vi "展开空白块.vi"(1 "索引":i32, 2 "地图":i16[][](array[numeric])) -> (0 "输出地图":i16[][](array[numeric]))   [LabVIEW 2017]
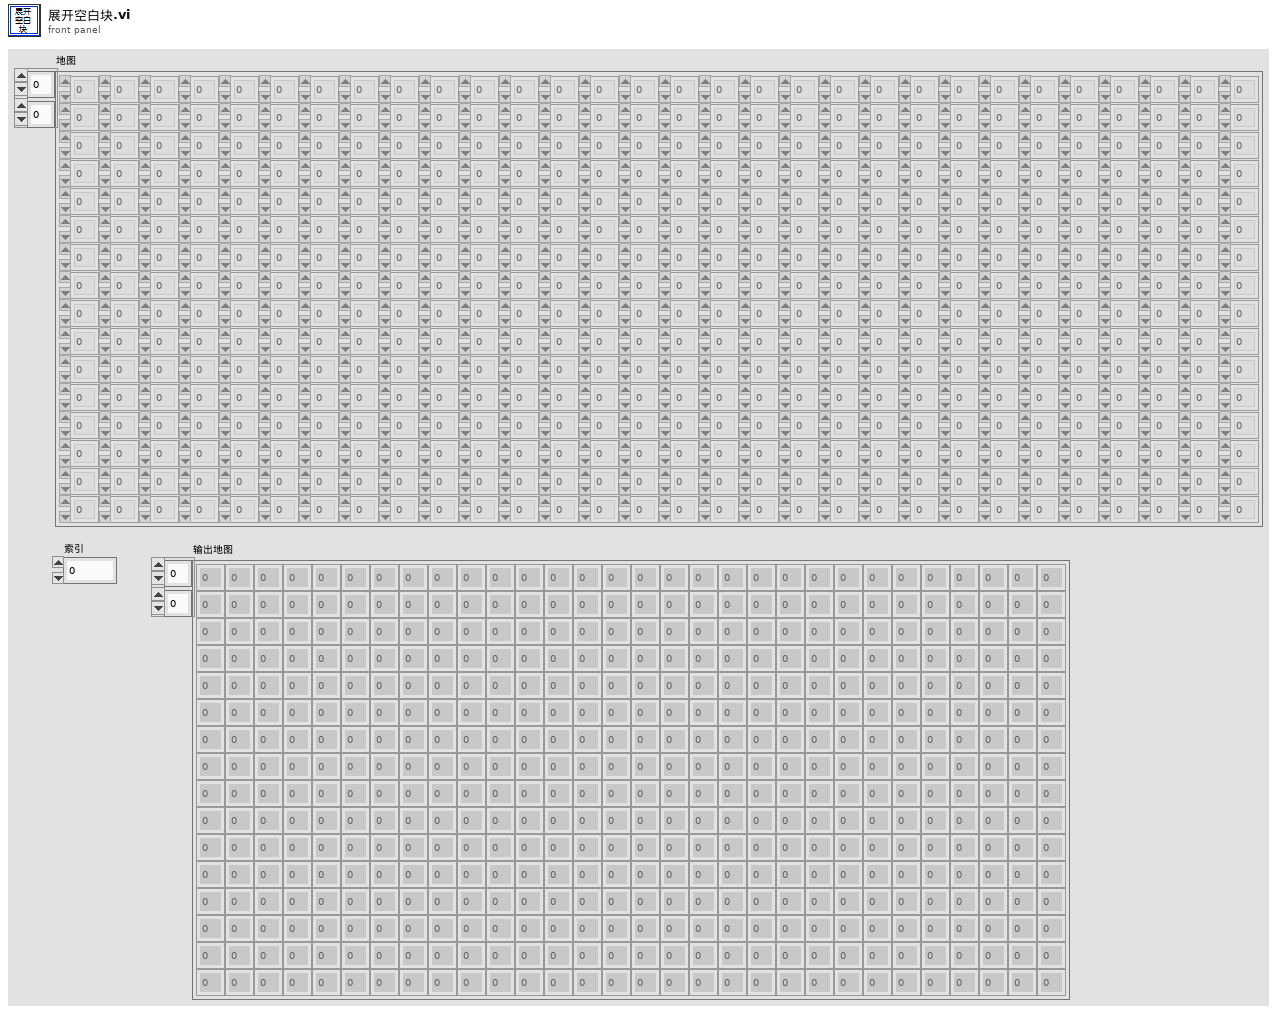
[diagram p1: front panel]
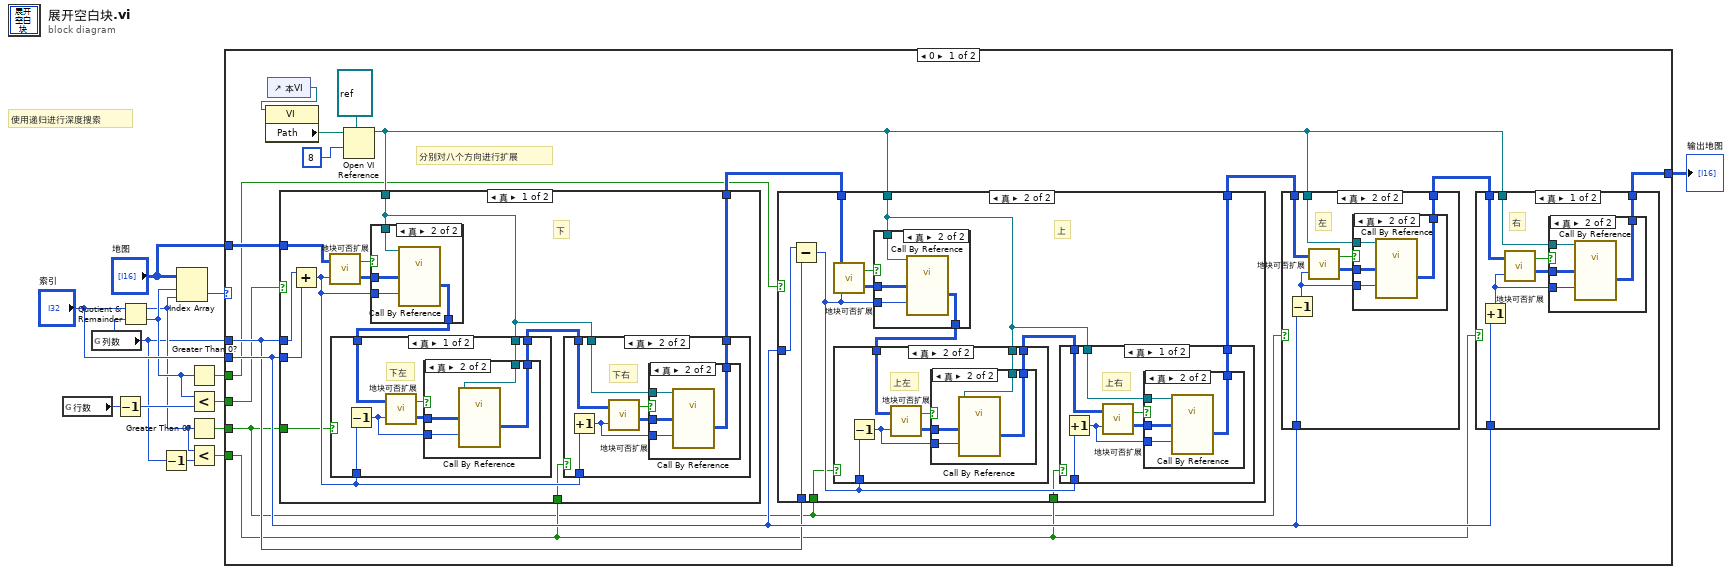
[diagram p0: block diagram]
diagram:
  # "使用递归进行深度搜索"
  n1 = global read "全局变量.vi" "行数"() -> (w10:i32)
  n2 = global read "全局变量.vi" "列数"() -> (w4:i32)
  n3 = Decrement(x=w10) -> (x-1=w9:i32)
  n4 = Quotient & Remainder(x="索引", y=w4) -> (x-y*floor(x/y)=w5:i32, floor(x/y)=w6:i32)
  n5 = Decrement(x=w4) -> (x-1=w3:i32)
  n6 = Index Array(array="地图", index (row)=w6, index (col)=w5) -> (element=w14:i16)
  n7 = Greater Than 0?(x=w6) -> (x > 0?=w7:bool)
  n8 = Less?(x=w6, y=w9) -> (x < y?=w8:bool)
  n9 = Greater Than 0?(x=w5) -> (x > 0?=w2:bool)
  n10 = Less?(x=w5, y=w3) -> (x < y?=w1:bool)
  n11 = case shown="0" w14 {
    tunnel: "索引" -> [w21 _]
    tunnel: "地图" -> [w20 w145]
    tunnel: [w27 w145] -> w12
    tunnel: w4 -> [w19 _]
    tunnel: w8 -> [w16 _]
    tunnel: w7 -> [w15 _]
    tunnel: w2 -> [w17 _]
    tunnel: w1 -> [w18 _]
    frame 0 {
      # "分别对八个方向进行扩展"
      n12 = control-ref of="本VI"() -> (w25:refnum<vi>)
      n13 = property class="VI"(reference=w25) -> ("Path"=w26:path)  [unwired: 1 in, 2 out]
      n14 = Open VI Reference(type specifier VI Refnum (for type only)=refnum<vi> refnum ("类型说明符VI引用句柄（仅用于类型）"), vi path=w26, options=8 ("选项")) -> (vi reference=w22:refnum<vi>)  [unwired: 3 in, 1 out]
      n15 = case shown="真" w16 {
        tunnel: w20 -> [w106 w144]
        tunnel: w21 -> [w112 _]
        tunnel: [w110 w144] -> w30
        tunnel: w22 -> [w104 _]
        tunnel: w19 -> [w103 _]
        tunnel: w18 -> [w102 _]
        tunnel: w17 -> [w101 _]
        frame True {
          # "下"
          n16 = Add(x=w103, y=w112) -> (x+y=w105:i32)
          n17 = call "地块可否扩展.vi"("索引"=w105, "地图"=w106) -> ("输出地图"=w108:i16[][], "可展开"=w107:bool)
          n18 = case shown="真" w107 {
            tunnel: w104 -> [_ w117]
            tunnel: [w113 w116] -> w109
            tunnel: w108 -> [w113 w115]
            tunnel: w105 -> [_ w114]
            frame False {
            }
            frame True {
              n19 = call-by-ref "?"(reference=w117, "索引"=w114, "地图"=w115) -> ("输出地图"=w116:i16[][])  [unwired: 1 in, 2 out]
            }
          }
          n20 = case shown="真" w101 {
            tunnel: w109 -> [w133 w143]
            tunnel: [w136 w143] -> w111
            tunnel: w104 -> [w137 _]
            tunnel: w105 -> [w131 _]
            frame True {
              # "下左"
              n21 = Decrement(x=w131) -> (x-1=w132:i32)
              n22 = call "地块可否扩展.vi"("索引"=w132, "地图"=w133) -> ("输出地图"=w135:i16[][], "可展开"=w134:bool)
              n23 = case shown="真" w134 {
                tunnel: w137 -> [_ w142]
                tunnel: w132 -> [_ w141]
                tunnel: w135 -> [w138 w140]
                tunnel: [w138 w139] -> w136
                frame False {
                }
                frame True {
                  n24 = call-by-ref "?"(reference=w142, "索引"=w141, "地图"=w140) -> ("输出地图"=w139:i16[][])  [unwired: 1 in, 2 out]
                }
              }
            }
            frame False {
            }
          }
          n25 = case shown="真" w102 {
            tunnel: w111 -> [w118 w119]
            tunnel: [w118 w124] -> w110
            tunnel: w105 -> [_ w125]
            tunnel: w104 -> [_ w123]
            frame False {
            }
            frame True {
              # "下右"
              n26 = Increment(x=w125) -> (x+1=w121:i32)
              n27 = call "地块可否扩展.vi"("索引"=w121, "地图"=w119) -> ("输出地图"=w122:i16[][], "可展开"=w120:bool)
              n28 = case shown="真" w120 {
                tunnel: w121 -> [_ w130]
                tunnel: w122 -> [w126 w129]
                tunnel: [w126 w128] -> w124
                tunnel: w123 -> [_ w127]
                frame False {
                }
                frame True {
                  n29 = call-by-ref "?"(reference=w127, "索引"=w130, "地图"=w129) -> ("输出地图"=w128:i16[][])  [unwired: 1 in, 2 out]
                }
              }
            }
          }
        }
        frame False {
        }
      }
      n30 = case shown="真" w15 {
        tunnel: w30 -> [w57 w63]
        tunnel: w21 -> [_ w68]
        tunnel: [w57 w67] -> w29
        tunnel: w22 -> [_ w61]
        tunnel: w17 -> [_ w60]
        tunnel: w18 -> [_ w59]
        tunnel: w19 -> [_ w58]
        frame False {
        }
        frame True {
          # "上"
          n31 = Subtract(x=w68, y=w58) -> (x-y=w62:i32)
          n32 = call "地块可否扩展.vi"("索引"=w62, "地图"=w63) -> ("输出地图"=w64:i16[][], "可展开"=w65:bool)
          n33 = case shown="真" w65 {
            tunnel: [w70 w74] -> w66
            tunnel: w61 -> [_ w73]
            tunnel: w64 -> [w70 w72]
            tunnel: w62 -> [_ w71]
            frame False {
            }
            frame True {
              n34 = call-by-ref "?"(reference=w73, "索引"=w71, "地图"=w72) -> ("输出地图"=w74:i16[][])  [unwired: 1 in, 2 out]
            }
          }
          n35 = case shown="真" w60 {
            tunnel: w66 -> [w88 w90]
            tunnel: [w88 w95] -> w69
            tunnel: w61 -> [_ w94]
            tunnel: w62 -> [_ w89]
            frame False {
            }
            frame True {
              # "上左"
              n36 = Decrement(x=w89) -> (x-1=w91:i32)
              n37 = call "地块可否扩展.vi"("索引"=w91, "地图"=w90) -> ("输出地图"=w92:i16[][], "可展开"=w93:bool)
              n38 = case shown="真" w93 {
                tunnel: [w96 w100] -> w95
                tunnel: w94 -> [_ w99]
                tunnel: w92 -> [w96 w98]
                tunnel: w91 -> [_ w97]
                frame False {
                }
                frame True {
                  n39 = call-by-ref "?"(reference=w99, "索引"=w97, "地图"=w98) -> ("输出地图"=w100:i16[][])  [unwired: 1 in, 2 out]
                }
              }
            }
          }
          n40 = case shown="真" w59 {
            tunnel: w69 -> [w78 w87]
            tunnel: w62 -> [w81 _]
            tunnel: [w80 w87] -> w67
            tunnel: w61 -> [w79 _]
            frame True {
              # "上右"
              n41 = Increment(x=w81) -> (x+1=w75:i32)
              n42 = call "地块可否扩展.vi"("索引"=w75, "地图"=w78) -> ("输出地图"=w76:i16[][], "可展开"=w77:bool)
              n43 = case shown="真" w77 {
                tunnel: [w82 w86] -> w80
                tunnel: w75 -> [_ w85]
                tunnel: w79 -> [_ w84]
                tunnel: w76 -> [w82 w83]
                frame False {
                }
                frame True {
                  n44 = call-by-ref "?"(reference=w84, "索引"=w85, "地图"=w83) -> ("输出地图"=w86:i16[][])  [unwired: 1 in, 2 out]
                }
              }
            }
            frame False {
            }
          }
        }
      }
      n45 = case shown="真" w17 {
        tunnel: w29 -> [w44 w48]
        tunnel: w21 -> [_ w51]
        tunnel: [w44 w49] -> w28
        tunnel: w22 -> [_ w50]
        frame False {
        }
        frame True {
          # "左"
          n46 = Decrement(x=w51) -> (x-1=w45:i32)
          n47 = call "地块可否扩展.vi"("索引"=w45, "地图"=w48) -> ("输出地图"=w46:i16[][], "可展开"=w47:bool)
          n48 = case shown="真" w47 {
            tunnel: w50 -> [_ w56]
            tunnel: [w52 w55] -> w49
            tunnel: w46 -> [w52 w54]
            tunnel: w45 -> [_ w53]
            frame False {
            }
            frame True {
              n49 = call-by-ref "?"(reference=w56, "索引"=w53, "地图"=w54) -> ("输出地图"=w55:i16[][])  [unwired: 1 in, 2 out]
            }
          }
        }
      }
      n50 = case shown="真" w18 {
        tunnel: w28 -> [w34 w43]
        tunnel: [w36 w43] -> w27
        tunnel: w21 -> [w37 _]
        tunnel: w22 -> [w35 _]
        frame True {
          # "右"
          n51 = Increment(x=w37) -> (x+1=w33:i32)
          n52 = call "地块可否扩展.vi"("索引"=w33, "地图"=w34) -> ("输出地图"=w32:i16[][], "可展开"=w31:bool)
          n53 = case shown="真" w31 {
            tunnel: [w38 w42] -> w36
            tunnel: w35 -> [_ w41]
            tunnel: w33 -> [_ w40]
            tunnel: w32 -> [w38 w39]
            frame False {
            }
            frame True {
              n54 = call-by-ref "?"(reference=w41, "索引"=w40, "地图"=w39) -> ("输出地图"=w42:i16[][])  [unwired: 1 in, 2 out]
            }
          }
        }
        frame False {
        }
      }
    }
    frame 1..8, Default {
    }
  }
  "输出地图" <- w12
